vi "Datalogging.vi"   [LabVIEW 2018]
uses:
  <vilib>/Rock Robotics/WPI/ThirdParty/Phoenix-LabVIEW/Motor Controller/Get/CTRE_Phoenix_MotorController_GetSelectedSensorData.vi
  Robot Global Data.vi
  <vilib>/Utility/file.llb/Write Delimited Spreadsheet (string).vi
types:
  T1 = typedef "WPI_MotorControlDeviceRef.ctl" = cluster{"DeviceStatus":errorcluster, "Type":T2, "PWM":cluster{"PWM Channel":T3, "DeadBand":T4}, "CAN":cluster{"Device Number":u8, "SetOutput VI Ref":variant, "GetOutput VI Ref":variant, "Enable VI Ref":variant, "Disable VI Ref":variant, "Data":variant}, "Invert":bool, "DIO PWM":cluster{"PWM \"Enable\" Channel":T3, "DIOChannel":T5, "PWM Rate":dbl}}
  T2 = typedef "WPI_MotorControlType.ctl" = enum16{"PWM", "CAN", "DIO PWM"}
  T3 = typedef "FPGA_DIOPWMChannel.ctl" = enum8{"PWM 0", "PWM 1", "PWM 2", "PWM 3", "PWM 4", "PWM 5", "PWM 6", "PWM 7", "PWM 8", "PWM 9", "PWM MXP 0", "PWM MXP 1", "PWM MXP 2", "PWM MXP 3", "PWM MXP 4", "PWM MXP 5", "PWM MXP 6", "PWM MXP 7", "PWM MXP 8", "PWM MXP 9", "Invalid"}
  T4 = typedef "WPI_PWMDeadband.ctl" = cluster{"Name":string, "maxPositivePwm":i32, "minPositivePwm":i32, "centerPwm":i32, "maxNegativePwm":i32, "minNegativePwm":i32, "angularRange":u16}
  T5 = typedef "FPGA_DIOChannel.ctl" = enum8{"DIO 0", "DIO 1", "DIO 2", "DIO 3", "DIO 4", "DIO 5", "DIO 6", "DIO 7", "DIO 8", "DIO 9", "DIO MXP 0", "DIO MXP 1", "DIO MXP 2", "DIO MXP 3", "DIO MXP 4", "DIO MXP 5", "DIO MXP 6", "DIO MXP 7", "DIO MXP 8", "DIO MXP 9", "DIO MXP 10", "DIO MXP 11", "DIO MXP 12", "DIO MXP 13", "DIO MXP 14", "DIO MXP 15", "SPI Port CS1", "SPI Port CS2", "SPI Port CS3", "SPI Port MISO", "SPI Port MOSI", "Invalid"}
  T6 = cluster{"Yaw":dbl, "Roll":dbl, "Pitch":dbl, "Heading":dbl, "Fused Heading":dbl}
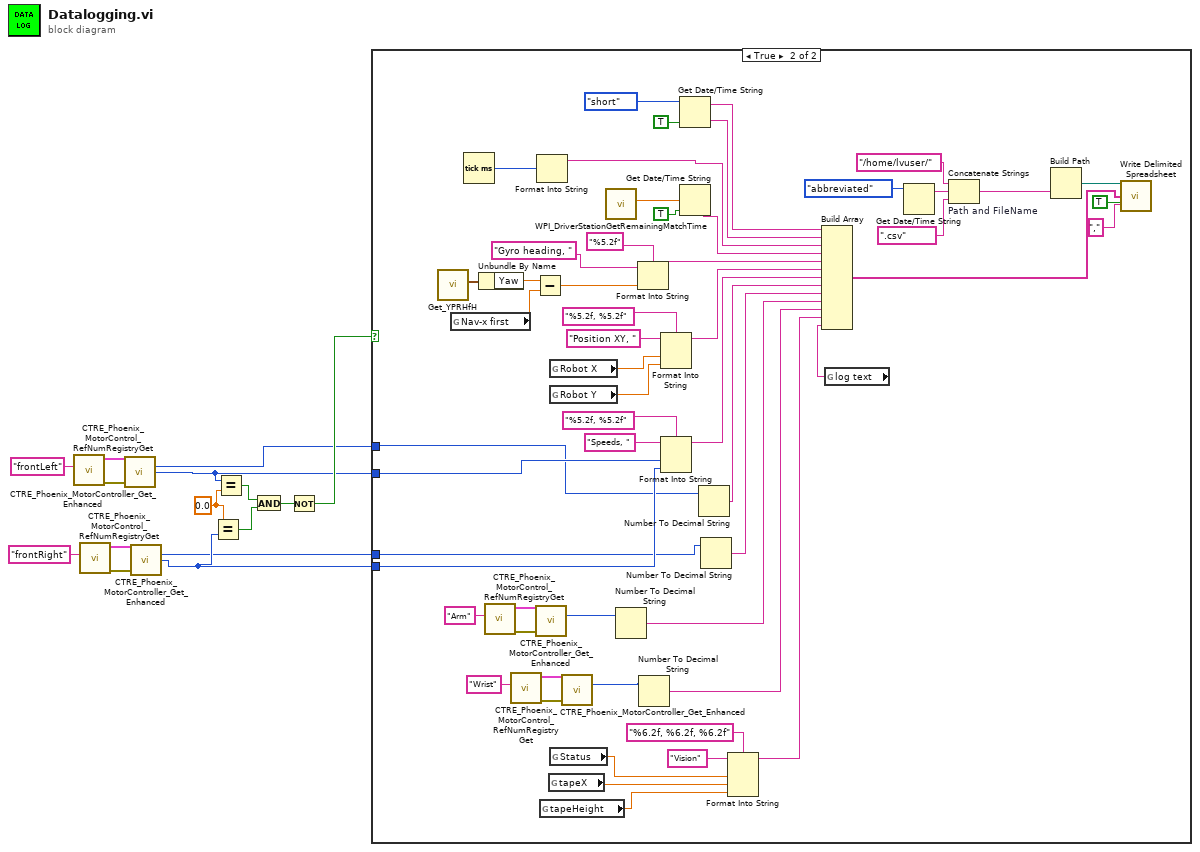
[diagram p0: block diagram]
diagram:
  w15 = 0.0 ("y")
  n1 = call <vilib>:"CTRE_Phoenix_MotorControl_RefNumRegistryGet.vi"("refnum name"="frontLeft") -> ("error out"=w10:errorcluster, "PhoenixMotorControlDevRef"=w9:T1)  [unwired: 9 in]
  n2 = call <vilib>:"CTRE_Phoenix_MotorControl_RefNumRegistryGet.vi"("refnum name"="frontRight") -> ("error out"=w6:errorcluster, "PhoenixMotorControlDevRef"=w5:T1)  [unwired: 9 in]
  n3 = call-poly <vilib>:"CTRE_Phoenix_MotorController_Get_Enhanced.vi"("PhoenixMotorControlDevRef"=w9, "error in"=w10) -> ("Position (Raw Sensor Units)"=w2:i32, "Velocity (Raw Sensor Units per 100 ms)"=w7:i32)  [unwired: 10 in, 2 out]
  n4 = call-poly <vilib>:"CTRE_Phoenix_MotorController_Get_Enhanced.vi"("PhoenixMotorControlDevRef"=w5, "error in"=w6) -> ("Position (Raw Sensor Units)"=w1:i32, "Velocity (Raw Sensor Units per 100 ms)"=w3:i32)  [unwired: 10 in, 2 out]
  n5 = Equal?(x=w15, y=w3) -> (x = y?=w13:bool)
  n6 = Equal?(x=w7, y=w15) -> (x = y?=w14:bool)
  n7 = And(x=w14, y=w13) -> (x .and. y?=w12:bool)
  n8 = Not(x=w12) -> (.not. x?=w11:bool)
  n9 = case shown="True" w11 {
    tunnel: w7 -> [_ w38]
    tunnel: w3 -> [_ w37]
    tunnel: w2 -> [_ w36]
    tunnel: w1 -> [_ w35]
    frame False {
    }
    frame True {
      n10 = call <vilib>:"Get_YPRHfH.vi"() -> ("YRPHfH"=w63:T6)  [unwired: 11 in]
      n11 = global read "Robot Global Data.vi" "Nav-x first"() -> (w71:dbl)
      n12 = Tick Count (ms)() -> (millisecond timer value=w40:u32)
      n13 = Unbundle By Name(w63) -> ("Yaw"=w64:dbl)
      n14 = call <vilib>:"CTRE_Phoenix_MotorControl_RefNumRegistryGet.vi"("refnum name"="Arm") -> ("error out"=w28:errorcluster, "PhoenixMotorControlDevRef"=w29:T1)  [unwired: 9 in]
      n15 = call <vilib>:"CTRE_Phoenix_MotorControl_RefNumRegistryGet.vi"("refnum name"="Wrist") -> ("error out"=w31:errorcluster, "PhoenixMotorControlDevRef"=w32:T1)  [unwired: 9 in]
      n16 = Subtract(x=w64, y=w71) -> (x-y=w61:dbl)
      n17 = call-poly <vilib>:"CTRE_Phoenix_MotorController_Get_Enhanced.vi"("PhoenixMotorControlDevRef"=w29, "error in"=w28) -> ("Position (Raw Sensor Units)"=w25:i32)  [unwired: 10 in, 3 out]
      n18 = Format Into String(w40) -> (resulting string=w39:string)  [unwired: 3 in, 1 out]
      n19 = global read "Robot Global Data.vi" "tapeHeight"() -> (w16:dbl)
      n20 = global read "Robot Global Data.vi" "tapeX"() -> (w17:dbl)
      n21 = global read "Robot Global Data.vi" "Robot X"() -> (w54:dbl)
      n22 = global read "Robot Global Data.vi" "Robot Y"() -> (w46:dbl)
      n23 = global read "Robot Global Data.vi" "Status"() -> (w18:dbl)
      n24 = call-poly <vilib>:"CTRE_Phoenix_MotorController_Get_Enhanced.vi"("PhoenixMotorControlDevRef"=w32, "error in"=w31) -> ("Position (Raw Sensor Units)"=w26:i32)  [unwired: 10 in, 3 out]
      n25 = call <vilib>:"WPI_DriverStationGetRemainingMatchTime.vi"() -> ("Match Time(s)"=w70:sgl)  [unwired: 10 in, 1 out]
      n26 = Number To Decimal String(number=w25) -> (decimal integer string=w24:string)  [unwired: 1 in]
      n27 = Format Into String(format string="%5.2f", initial string="Gyro heading, " ("element"), w61) -> (resulting string=w43:string)  [unwired: 1 in, 1 out]
      n28 = Number To Decimal String(number=w26) -> (decimal integer string=w23:string)  [unwired: 1 in]
      n29 = Format Into String(format string="%5.2f, %5.2f", initial string="Position XY, ", w54, w46) -> (resulting string=w42:string)  [unwired: 1 in, 1 out]
      n30 = Format Into String(format string="%5.2f, %5.2f", initial string="Speeds, ", w38, w37) -> (resulting string=w41:string)  [unwired: 1 in, 1 out]
      n31 = Get Date/Time String(date format (0)=enum16{"short", "long", "abbreviated"}."short", want seconds? (F)=TRUE) -> (date string=w53:string, time string=w52:string)  [unwired: 1 in]
      n32 = Get Date/Time String(seconds (now)=w70, want seconds? (F)=TRUE) -> (time string=w65:string)  [unwired: 1 in, 1 out]
      n33 = Number To Decimal String(number=w36) -> (decimal integer string=w34:string)  [unwired: 1 in]
      n34 = Number To Decimal String(number=w35) -> (decimal integer string=w33:string)  [unwired: 1 in]
      n35 = Format Into String(format string="%6.2f, %6.2f, %6.2f", initial string="Vision", w18, w17, w16) -> (resulting string=w20:string)  [unwired: 1 in, 1 out]
      n36 = global read "Robot Global Data.vi" "log text"() -> (w19:string)
      n37 = Build Array(w53, w52, w39, w65, w43, w42, w41, w34, w33, w24, w23, w20, w19) -> (w68:string[])
      n38 = Get Date/Time String(date format (0)=enum16{"short", "long", "abbreviated"}."abbreviated") -> (date string=w55:string)  [unwired: 2 in, 1 out]
      n39 = Concatenate Strings "Path and FileName"("/home/lvuser/", w55, ".csv") -> (w58:string)
      n40 = Build Path(name or relative path=w58) -> (appended path=w57:path)  [unwired: 1 in]
      n41 = call-poly <vilib>:"Write Delimited Spreadsheet.vi"("file path (dialog if empty)"=w57, "1D data"=w68, "append to file? (new file:F)"=TRUE, "delimiter (\\t)"="," ("delimiter (\\t)")) -> ()  [unwired: 10 in, 2 out]
    }
  }
